vi "Variant_GetType.vi"(11 "Variant":variant) -> (1 "Type Enum":T1=enum."String" format="0x%02x", 2 "Type":u8 format="%.0x", 3 "Variant dup":variant)   [LabVIEW 2013, in "OpenVariant.lvlib"]
uses:
  OpenVariant.lvlib
  <vilib>/Utility/GetType.llb/Type Enum.ctl
  <vilib>/Utility/VariantDataType/TypedefInfo.ctl
  TypeDescriptor/OpenDescriptor.lvlib
  <vilib>/Utility/VariantDataType/VariantType.lvlib
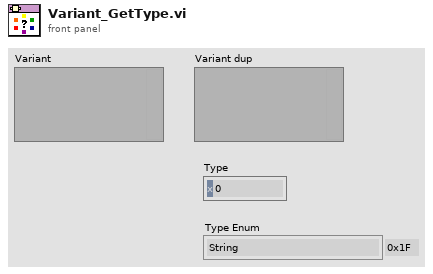
[diagram p1: front panel]
types:
  T1 = typedef "Type Enum.ctl" = enum8{"Void", "I8", "I16", "I32", "I64", "U8", "U16", "U32", "U64", "Single Float", "Double Float", "Extended Float", "Single Complex", "Double Complex", "Extended Complex", "Enum I8 NEVER", "Enum I16 NEVER", "Enum I32 NEVER", "Enum I64 NEVER", "Enum U8", "Enum U16", "Enum U32", "Enum U64", "Single Float With Unit", "Double Float With Unit", "Extended Float With Unit", "Single Complex With Unit", "Double Complex With Unit", "Extended Complex With Unit", "boolU16", "Boolean", "String", "Handle", "Path", "Picture", "C String", "Pascal String", "Tag", "SubString", "Array", "SubArray", "Cluster", "Numeric Cluster", "Variant", "LV Variant", "Measure Data (waveform)", "Refnum", "ExtData", "function", "Typedef", "Poly VI", "bad wire", "LabVIEW Class Instance"}
  T2 = typedef "VariantType.lvlib/TypedefInfo.ctl" = cluster{"Name":string, "Timestamp":u32}
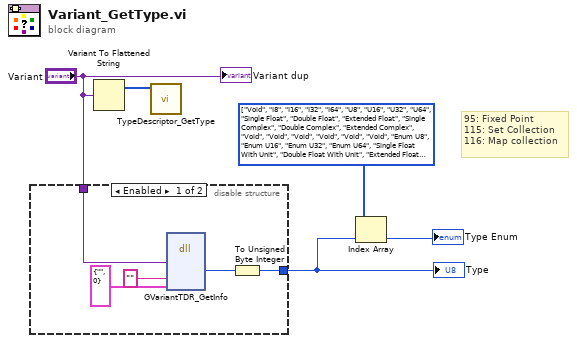
[diagram p0: block diagram]
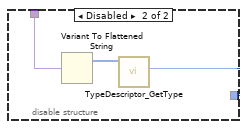
[diagram p2: hidden frame]
diagram:
  w3 = T1[] [enum."Void", enum."I8", enum."I16", enum."I32", enum."I64", enum."U8", enum."U16", enum."U32", enum."U64", enum."Single Float", enum."Double Float", enum."Extended Float", enum."Single Complex", enum."Double Complex", enum."Extended Complex", enum."Void", enum."Void", enum."Void", enum."Void", enum."Void", enum."Void", enum."Enum U8", enum."Enum U16", enum."Enum U32", enum."Enum U64", enum."Single Float With Unit", enum."Double Float With Unit", enum."Extended Float With Unit", enum."Single Complex With Unit", enum."Double Complex With Unit", enum."Extended Complex With Unit", enum."Void", enum."Void", enum."Boolean", enum."Void", enum."Void", enum."Void", enum."Void", enum."Void", enum."Void", enum."Void", enum."Void", enum."Void", enum."Void", enum."Void", enum."Void", enum."Void", enum."Void", enum."String", enum."Void", enum."Path", enum."Picture", enum."Void", enum."Void", enum."Void", enum."Tag", enum."Void", enum."Void", enum."Void", enum."Void", enum."Void", enum."Void", enum."Void", enum."Void", enum."Array", enum."Void", enum."Void", enum."Void", enum."Void", enum."Void", enum."Void", enum."Void", enum."Void", enum."Void", enum."Void", enum."Void", enum."Void", enum."Void", enum."Void", enum."Array", enum."Cluster", enum."Void", enum."Variant", enum."LV Variant", enum."Measure Data (waveform)", enum."Void", enum."Void", enum."Void", enum."Void", enum."Void", enum."Void", enum."Void", enum."Void", enum."Void", enum."Void", enum."Void", enum."Void", enum."Void", enum."Void", enum."Void", enum."Void", enum."Void", enum."Void", enum."Void", enum."Void", enum."Void", enum."Void", enum."Void", enum."Void", enum."Void", enum."Void", enum."Void", enum."Refnum", enum."Void", enum."Void", enum."Void", enum."Void", enum."Void", enum."Void", enum."Void", enum."Void", enum."Void", enum."Void", enum."Void", enum."Void", enum."Void", enum."Void", enum."Void", enum."Void", enum."Void", enum."Void", enum."Void", enum."ExtData", enum."Void", enum."Void", enum."Void", enum."Void", enum."Void", enum."Void", enum."Void", enum."Void", enum."Void", enum."Void", enum."Void", enum."Void", enum."Void", enum."Void", enum."Void", enum."Void", enum."Void", enum."Void", enum."Void", enum."Void", enum."Void", enum."Void", enum."Void", enum."Void", enum."Void", enum."Void", enum."Void", enum."Void", enum."Void", enum."Void", enum."Void", enum."Void", enum."Void", enum."Void", enum."Void", enum."Void", enum."Void", enum."Void", enum."Void", enum."Void", enum."Void", enum."Void", enum."Void", enum."Void", enum."Void", enum."Void", enum."Void", enum."Void", enum."Void", enum."Void", enum."Void", enum."Void", enum."Void", enum."Void", enum."Void", enum."Void", enum."Void", enum."Void", enum."Void", enum."Void", enum."Void", enum."Void", enum."Void", enum."Void", enum."Void", enum."Void", enum."Void", enum."Void", enum."Void", enum."Void", enum."Void", enum."Void", enum."Void", enum."Void", enum."Void", enum."Void", enum."Void", enum."Void", enum."Void", enum."Void", enum."Void", enum."Void", enum."Void", enum."Void", enum."Void", enum."Void", enum."Void", enum."Void", enum."Void", enum."Void", enum."Void", enum."Void", enum."Void", enum."Void", enum."Void", enum."Void", enum."Void", enum."Void", enum."Void", enum."Void", enum."Void", enum."Void", enum."Void", enum."Void", enum."Void", enum."Void", enum."Void", enum."function", enum."Void", enum."Poly VI", enum."Void", enum."Void", enum."Void", enum."Void", enum."Void", enum."Void", enum."Void", enum."Void", enum."Void", enum."Void", enum."Void", enum."Void", enum."Void"] items=["Void", "I8", "I16", "I32", "I64", "U8", "U16", "U32", "U64", "Single Float", "Double Float", "Extended Float", "Single Complex", "Double Complex", "Extended Complex", "Enum I8 NEVER", "Enum I16 NEVER", "Enum I32 NEVER", "Enum I64 NEVER", "Enum U8", "Enum U16", "Enum U32", "Enum U64", "Single Float With Unit", "Double Float With Unit", "Extended Float With Unit", "Single Complex With Unit", "Double Complex With Unit", "Extended Complex With Unit", "boolU16", "Boolean", "String", "Handle", "Path", "Picture", "C String", "Pascal String", "Tag", "SubString", "Array", "SubArray", "Cluster", "Numeric Cluster", "Variant", "LV Variant", "Measure Data (waveform)", "Refnum", "ExtData", "function", "Typedef", "Poly VI", "bad wire", "LabVIEW Class Instance"]
  # "95: Fixed Point\n115: Set Collection\n116: Map collection"
  n1 = disable-structure shown="Enabled" {
    disable-tunnel: "Variant" -> [w8 w13]
    disable-tunnel: [w6 w11] -> w1
    frame Enabled {
      n2 = dll-call lib="LabVIEW" fn="GVariantTDR_GetInfo"("lvVar"=w8, "name"="", "typeDef"=T2 {"Name"="", "Timestamp"=0} ("TypedefInfo")) -> ("typeCode"=w7:i16)  [unwired: 4 in, 6 out]
      n3 = To Unsigned Byte Integer(number=w7) -> (unsigned 8bit integer=w6:u8)
    }
    frame Disabled {
      n4 = Variant To Flattened String(Variant=w13) -> (1:w12:i16[])  [unwired: 1 out]
      n5 = call "TypeDescriptor_GetType.vi"("type descriptor"=w12) -> ("Type"=w11:u8)  [unwired: 9 in, 1 out]
    }
  }
  "Type" <- w1
  n6 = Variant To Flattened String(Variant="Variant") -> (1:w5:i16[])  [unwired: 1 out]
  n7 = call "TypeDescriptor_GetType.vi"("type descriptor"=w5) -> ()  [unwired: 9 in, 2 out]
  n8 = Index Array(array=w3, index=w1) -> (element=→"Type Enum":T1)
  "Variant dup" <- "Variant"
